vi "tags array to map.vi"(11 "channel tags":cluster{"key":string, "value":string}[](array[cluster])) -> (3 "map":map{string, string}(c390))   [LabVIEW 2020, in "nominal core steps.lvlib"]
doc: "Simple helper to convert a tag array to a map\n\n%docs-exclude%"
uses:
  nominal core steps.lvlib
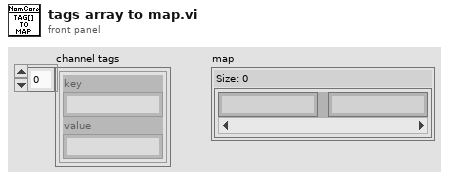
[diagram p1: front panel]
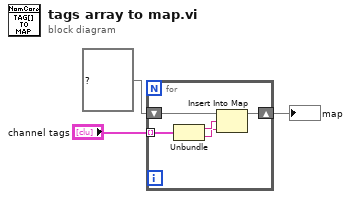
[diagram p0: block diagram]
diagram:
  n1 = for {
    tunnel: "channel tags" -> [w8] mode=indexing
    shift-right: [w5] -> w3
    shift-left: map{string, string} {} ("map") -> [w6]
    n2 = Unbundle(w8) -> ("key"=w7:string, "value"=w4:string)
    n3 = Insert Into Map(map in=w6, key=w7, value=w4) -> (map out=w5:map{string, string})  [unwired: 2 out]
  }
  "map" <- w3
